vi "GlobalMenuStatusStorage2.vi"() -> ()   [LabVIEW 2025]
panel:
  in  "Cluster":T1
  in  "?":enum32{"Scheduling"}(tab)
  out "Storyline":string
  in  "Power for each agent":enum32{"Gen", "DESD", "PV", "WT", "Load"}(tab)
  in  "Power for Generator":enum32{"Gen 1", "Gen 2"}(tab)
  out "Gen1 Power":cluster{dbl[], "gen1":dbl[]}(graph)
  out "Gen2 Power":cluster{dbl[], "gen2":dbl[]}(graph)
  in  "Power for DESD Battery":enum32{"DESD 1", "DESD 2", "DESD 3", "DESD 4"}(tab)
  out "DESD1 Power":cluster{dbl[], "desd1":dbl[]}(graph)
  out "DESD2 Power":cluster{dbl[], "desd2":dbl[]}(graph)
  out "DESD3 Power":cluster{dbl[], "desd3":dbl[]}(graph)
  out "DESD4 Power":cluster{dbl[], "desd4":dbl[]}(graph)
  in  "Power for Photovoltaic":enum32{"PV 1", "PV 2"}(tab)
  out "PV1 Power":cluster{dbl[], "pv1":dbl[]}(graph)
  out "PV2 Power":cluster{dbl[], "pv2":dbl[]}(graph)
  out "WT Power":cluster{dbl[], "wt1":dbl[]}(graph)
  in  "Power for Load":T2(tab)
  out "Load1 Power":cluster{dbl[], "load1":dbl[]}(graph)
  out "Load2 Power":cluster{dbl[], "load2":dbl[]}(graph)
  out "Load3 Power":cluster{dbl[], "load3":dbl[]}(graph)
  out "Load4 Power":cluster{dbl[], "load4":dbl[]}(graph)
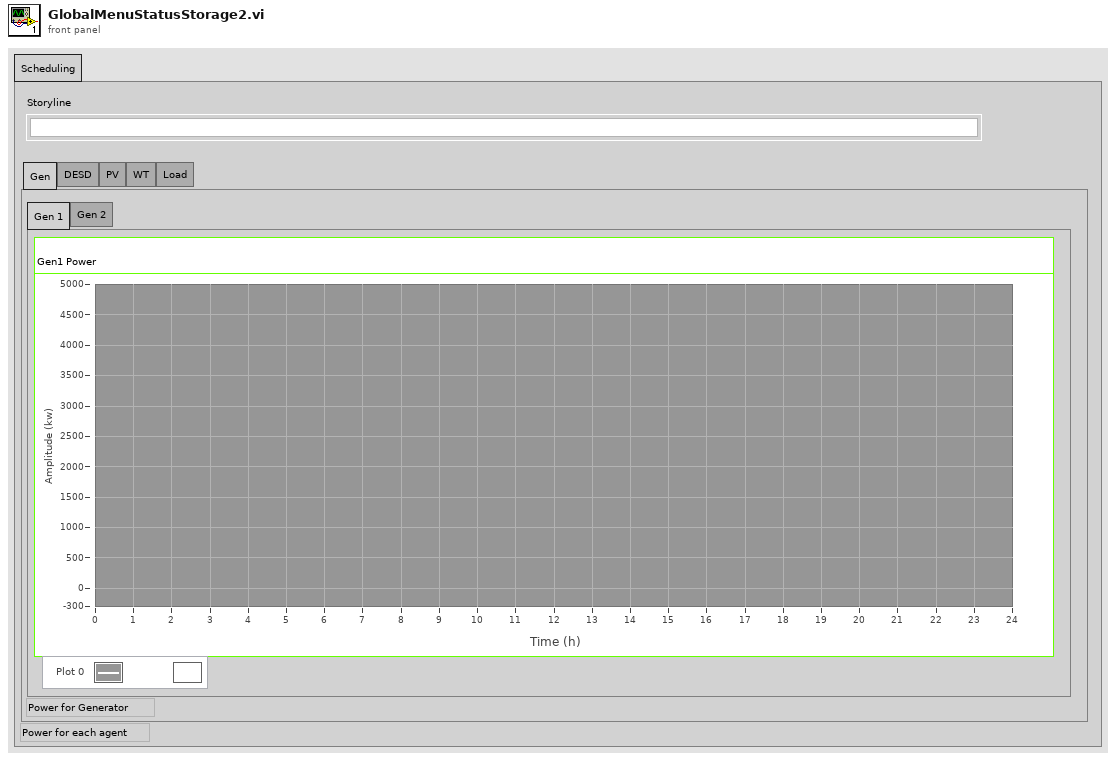
[diagram p1: front panel]
types:
  T1 = cluster{"time":dbl[], "gen1":dbl[], "gen2":dbl[], "desd1":dbl[], "desd2":dbl[], "desd3":dbl[], "desd4":dbl[], "pv1":dbl[], "pv2":dbl[], "wt1":dbl[], "load1":dbl[], "load2":dbl[], "load3":dbl[], "load4":dbl[], "type":string, "event":string}
  T2 = enum32{"Load 1", "Load 2(Hospital)", "Load 3", "Load 4(Comm Center)"}
  T3 = cluster{"time":dbl[], "gen1":dbl[], "gen2":dbl[], "desd1":dbl[], "desd2":dbl[], "desd3":dbl[], "desd4":dbl[], "pv1":dbl[], "pv2":dbl[], "wt1":dbl[], "load1":dbl[], "load2":dbl[], "load3":dbl[], "load4":dbl[]}
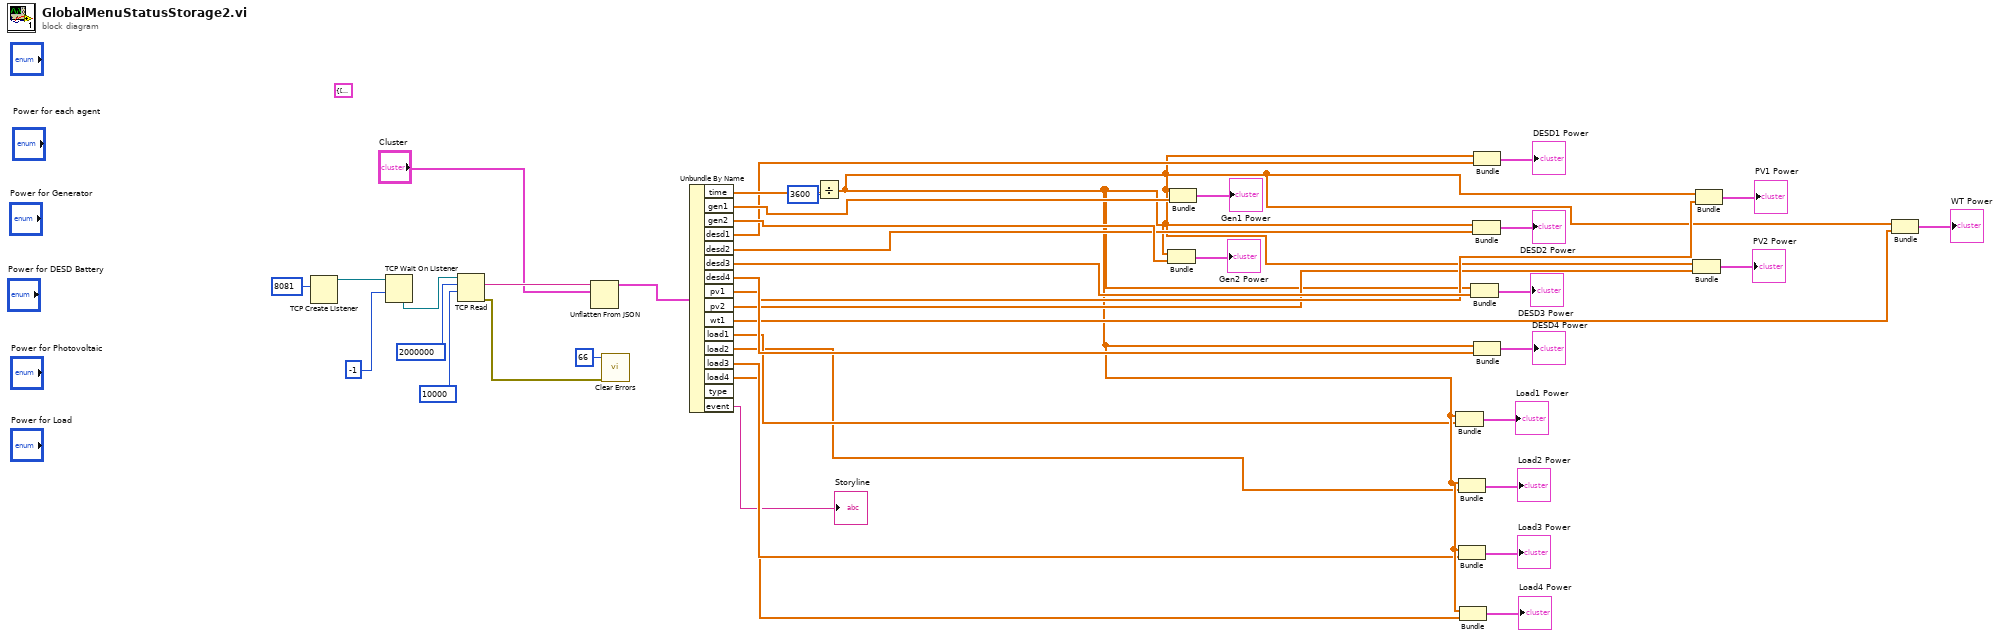
[diagram p0: block diagram]
diagram:
  (unwired) T3 {"time"=[], "gen1"=[], "gen2"=[], "desd1"=[], "desd2"=[], "desd3"=[], "desd4"=[], "pv1"=[], "pv2"=[], "wt1"=[], "load1"=[], "load2"=[], "load3"=[], "load4"=[]} ("Cluster")
  n1 = TCP Create Listener(10:u16 8081 ("port")) -> (3:w39:refnum<k5>)  [unwired: 4 in, 2 out]
  n2 = TCP Wait On Listener(9:-1 ("timeout ms (wait forever: -1)"), 11:w39) -> (4:w38:refnum<k5>)  [unwired: 2 in, 4 out]
  n3 = TCP Read(connection ID=w38, bytes to read=2000000, 9:10000 ("timeout ms (25000)")) -> (data out=w31:string, error out=w35:errorcluster)  [unwired: 2 in, 1 out]
  n4 = Unflatten From JSON(JSON string=w31, type and defaults="Cluster") -> (value=w33:T1)  [unwired: 5 in, 1 out]
  n5 = call <vilib>:"Clear Errors.vi"("error in (no error)"=w35, "specific error code to clear (0: all)"=66) -> ()  [unwired: 4 in, 2 out]
  n6 = Unbundle By Name(w33) -> ("time"=w29:dbl[], "gen1"=w32:dbl[], "gen2"=w26:dbl[], "desd1"=w21:dbl[], "desd2"=w20:dbl[], "desd3"=w19:dbl[], "desd4"=w18:dbl[], "pv1"=w15:dbl[], "pv2"=w14:dbl[], "wt1"=w12:dbl[], "load1"=w6:dbl[], "load2"=w5:dbl[], "load3"=w4:dbl[], "load4"=w3:dbl[], "event"=→"Storyline":string)  [unwired: 1 out]
  n7 = Divide(x=w29, y=3600) -> (x/y=w7:dbl[])
  n8 = Bundle(w7, "gen2"=w26) -> (→"Gen2 Power":cluster{dbl[], "gen2":dbl[]})  [unwired: 1 in]
  n9 = Bundle(w7, "gen1"=w32) -> (→"Gen1 Power":cluster{dbl[], "gen1":dbl[]})  [unwired: 1 in]
  n10 = Bundle(w7, "load1"=w6) -> (→"Load1 Power":cluster{dbl[], "load1":dbl[]})  [unwired: 1 in]
  n11 = Bundle(w7, "load2"=w5) -> (→"Load2 Power":cluster{dbl[], "load2":dbl[]})  [unwired: 1 in]
  n12 = Bundle(w7, "load3"=w4) -> (→"Load3 Power":cluster{dbl[], "load3":dbl[]})  [unwired: 1 in]
  n13 = Bundle(w7, "load4"=w3) -> (→"Load4 Power":cluster{dbl[], "load4":dbl[]})  [unwired: 1 in]
  n14 = Bundle(w7, "desd3"=w19) -> (→"DESD3 Power":cluster{dbl[], "desd3":dbl[]})  [unwired: 1 in]
  n15 = Bundle(w7, "desd2"=w20) -> (→"DESD2 Power":cluster{dbl[], "desd2":dbl[]})  [unwired: 1 in]
  n16 = Bundle(w7, "desd1"=w21) -> (→"DESD1 Power":cluster{dbl[], "desd1":dbl[]})  [unwired: 1 in]
  n17 = Bundle(w7, "desd4"=w18) -> (→"DESD4 Power":cluster{dbl[], "desd4":dbl[]})  [unwired: 1 in]
  n18 = Bundle(w7, "pv2"=w14) -> (→"PV2 Power":cluster{dbl[], "pv2":dbl[]})  [unwired: 1 in]
  n19 = Bundle(w7, "pv1"=w15) -> (→"PV1 Power":cluster{dbl[], "pv1":dbl[]})  [unwired: 1 in]
  n20 = Bundle(w7, "wt1"=w12) -> (→"WT Power":cluster{dbl[], "wt1":dbl[]})  [unwired: 1 in]
